vi "Tag_Value_Entry_PopUp.vi"(6 "Write Type":enum16{"SetRequest", "WriteValue"}(ring), 7 "Namespace":string, 8 "error in (no error)":errorcluster, 9 "Timeout (-1)":i32=-1, 10 "Synchronous (F)":bool, 11 "Tag Name":string) -> (0 "error out":errorcluster, 1 "found":bool, 2 "New Value":variant, 3 "Apply":bool)   [LabVIEW 2020, in "Tag Watchlist.lvlib"]
doc: "Tag value entrry pop-up. By specifying a Tag Name, the tag's value is looked up and the appropriately typed popup is launched.\n\nSelect either SetRequest or WriteValue for Write Type. Write value should be for debugging and testing purposes only. Set Request send the value by Set Request event instead of writing directly to the Tag's value.\n\nSupported Types are:\n- Boolean\n- Signed Integer\n- Unsigned Integer\n- Floating Point\n- String\n\nAny other type will launch the string value entry popup with the JSON representation of the value. BE CAREFUL."
uses:
  Tag Watchlist.lvlib
  Tag Engine.lvlib
  Tag/Tag.lvclass
  <vilib>/JDP Science/JSONtext/JSONtext.lvlib
panel:
  # "!!! Write Value is for debugging purposes only !!"
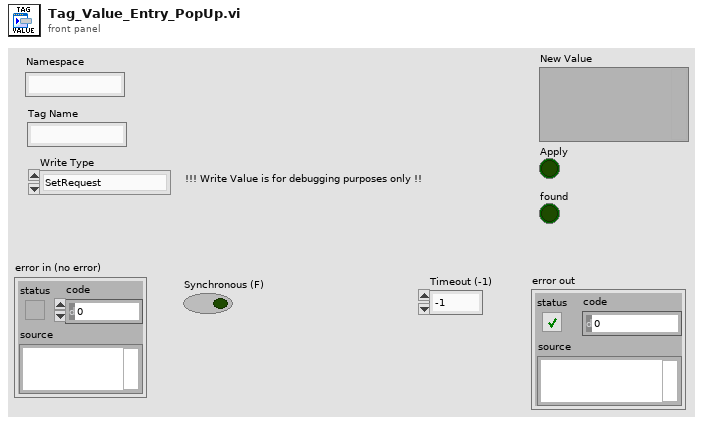
[diagram p1: front panel]
types:
  T1 = typedef "NI_Data Type.lvlib/Data Type.ctl" = enum8{"Invalid Type", "Void", "I8", "I16", "I32", "I64", "U8", "U16", "U32", "U64", "Single Float", "Double Float", "Extended Float", "Single Complex", "Double Complex", "Extended Complex", "Enum U8", "Enum U16", "Enum U32", "Enum U64", "Single Float With Unit", "Double Float With Unit", "Extended Float With Unit", "Single Complex with Unit", "Double Complex with Unit", "Extended Complex with Unit", "Boolean", "String", "Path", "Picture", "Tag", "Array", "Cluster", "Variant", "LV Variant", "Waveform", "Timestamp", "Digital Waveform", "Digital Data", "ExpressData", "Refnum", "External Data", "VI", "Poly VI", "LabVIEW Class Instance", "Fixed Point", "Set Collection", "Map Collection"}
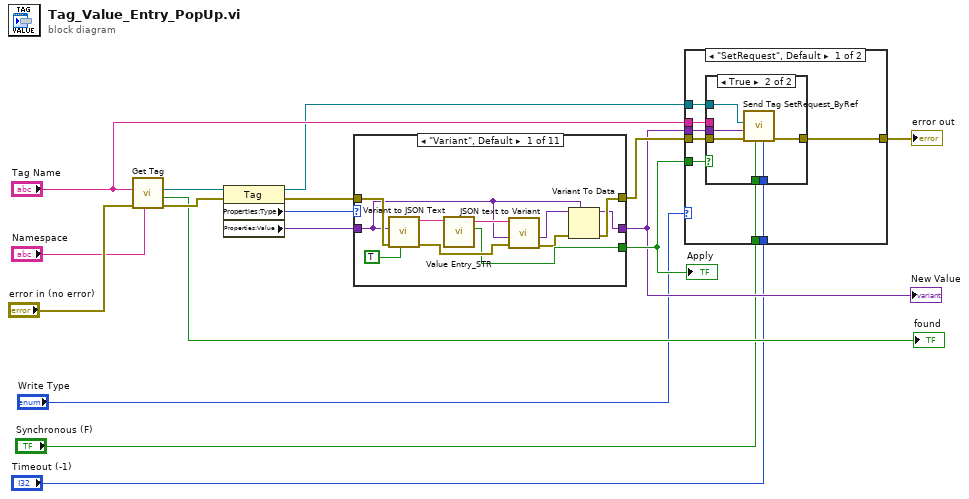
[diagram p0: block diagram]
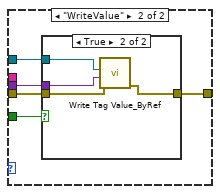
[diagram p3: hidden frame]
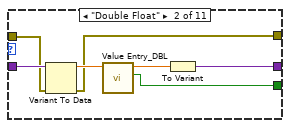
[diagram p5: hidden frame]
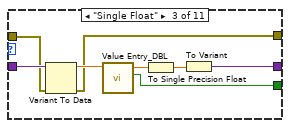
[diagram p6: hidden frame]
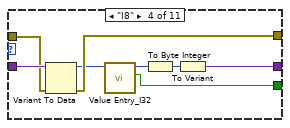
[diagram p7: hidden frame]
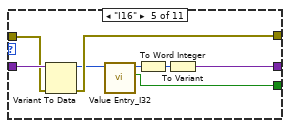
[diagram p8: hidden frame]
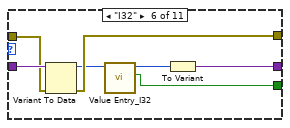
[diagram p9: hidden frame]
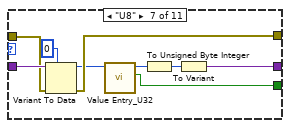
[diagram p10: hidden frame]
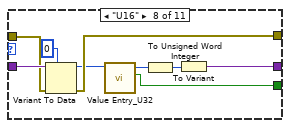
[diagram p11: hidden frame]
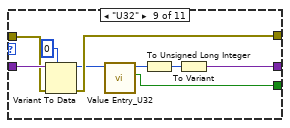
[diagram p12: hidden frame]
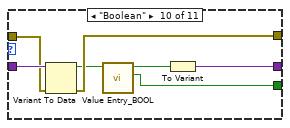
[diagram p13: hidden frame]
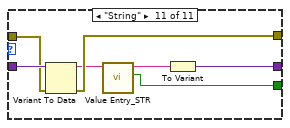
[diagram p14: hidden frame]
diagram:
  n1 = call "Get Tag.vi"("Namespace"="Namespace", "error in (no error)"="error in (no error)", "Name"="Tag Name") -> ("error out"=w7:errorcluster, "found"=→"found":bool, "Tag Ref out"=w17:refnum<data-value>)  [unwired: 6 in]
  n2 = property class="Tag"(reference=w17, error in=w7) -> (reference out=w4:refnum<data-value>, error out=w13:errorcluster, "Properties:Type"=w16:T1, "Properties:Value"=w15:variant)
  n3 = case shown="\"Variant\", Default" w16 {
    tunnel: w15 -> [w20 w35 w43 w51 w59 w66 w75 w84 w93 w100 w107]
    tunnel: w13 -> [w24 w33 w41 w50 w58 w65 w74 w83 w92 w99 w106]
    tunnel: [w21 w32 w40 w49 w57 w64 w73 w82 w91 w98 w105] -> w12
    tunnel: [w23 w30 w39 w46 w54 w61 w70 w79 w88 w94 w101] -> w11
    tunnel: [w19 w29 w38 w48 w56 w63 w72 w81 w90 w97 w104] -> w9
    frame "Variant", Default {
      n4 = call <vilib>:"Variant to JSON Text.vi"("Pretty Print?"=TRUE, "error in (no error)"=w24, "Variant"=w20) -> ("error out"=w25:errorcluster, "<JSON>"=w27:string)  [unwired: 6 in, 1 out]
      n5 = call "Value Entry_STR.vi"("Value In"=w27) -> ("Apply"=w23:bool, "Value Out"=w26:string)  [unwired: 9 in]
      n6 = call <vilib>:"JSON text to Variant.vi"("error in (no error)"=w25, "Data Type"=w20, "JSON"=w26) -> ("error out"=w22:errorcluster, "Variant out"=w18:variant)  [unwired: 7 in]
      n7 = Variant To Data(error in=w22, type=w20, Variant=w18) -> (data=w19:variant, error out=w21:errorcluster)
    }
    frame "Double Float" {
      n8 = Variant To Data(error in=w33, Variant=w35) -> (data=w34:dbl, error out=w32:errorcluster)  [unwired: 1 in]
      n9 = call "Value Entry_DBL.vi"("Value In"=w34) -> ("Apply"=w30:bool, "Value Out"=w31:dbl)  [unwired: 9 in]
      n10 = To Variant(anything=w31) -> (Variant=w29:variant)
    }
    frame "Single Float" {
      n11 = Variant To Data(error in=w41, Variant=w43) -> (data=w42:dbl, error out=w40:errorcluster)  [unwired: 1 in]
      n12 = call "Value Entry_DBL.vi"("Value In"=w42) -> ("Apply"=w39:bool, "Value Out"=w37:dbl)  [unwired: 9 in]
      n13 = To Single Precision Float(number=w37) -> (single precision float=w36:sgl)
      n14 = To Variant(anything=w36) -> (Variant=w38:variant)
    }
    frame "I8" {
      n15 = Variant To Data(error in=w50, Variant=w51) -> (data=w47:i32, error out=w49:errorcluster)  [unwired: 1 in]
      n16 = call "Value Entry_I32.vi"("Value In"=w47) -> ("Apply"=w46:bool, "Value Out"=w45:i32)  [unwired: 9 in]
      n17 = To Byte Integer(number=w45) -> (8bit integer=w44:i8)
      n18 = To Variant(anything=w44) -> (Variant=w48:variant)
    }
    frame "I16" {
      n19 = Variant To Data(error in=w58, Variant=w59) -> (data=w55:i32, error out=w57:errorcluster)  [unwired: 1 in]
      n20 = call "Value Entry_I32.vi"("Value In"=w55) -> ("Apply"=w54:bool, "Value Out"=w53:i32)  [unwired: 9 in]
      n21 = To Word Integer(number=w53) -> (16bit integer=w52:i16)
      n22 = To Variant(anything=w52) -> (Variant=w56:variant)
    }
    frame "I32" {
      n23 = Variant To Data(error in=w65, Variant=w66) -> (data=w62:i32, error out=w64:errorcluster)  [unwired: 1 in]
      n24 = call "Value Entry_I32.vi"("Value In"=w62) -> ("Apply"=w61:bool, "Value Out"=w60:i32)  [unwired: 9 in]
      n25 = To Variant(anything=w60) -> (Variant=w63:variant)
    }
    frame "U8" {
      n26 = Variant To Data(error in=w74, type=u32 0, Variant=w75) -> (data=w71:u32, error out=w73:errorcluster)
      n27 = call "Value Entry_U32.vi"("Value In"=w71) -> ("Apply"=w70:bool, "Value Out"=w67:u32)  [unwired: 9 in]
      n28 = To Unsigned Byte Integer(number=w67) -> (unsigned 8bit integer=w68:u8)
      n29 = To Variant(anything=w68) -> (Variant=w72:variant)
    }
    frame "U16" {
      n30 = Variant To Data(error in=w83, type=u32 0, Variant=w84) -> (data=w80:u32, error out=w82:errorcluster)
      n31 = call "Value Entry_U32.vi"("Value In"=w80) -> ("Apply"=w79:bool, "Value Out"=w77:u32)  [unwired: 9 in]
      n32 = To Unsigned Word Integer(number=w77) -> (unsigned 16bit integer=w76:u16)
      n33 = To Variant(anything=w76) -> (Variant=w81:variant)
    }
    frame "U32" {
      n34 = Variant To Data(error in=w92, type=u32 0, Variant=w93) -> (data=w89:u32, error out=w91:errorcluster)
      n35 = call "Value Entry_U32.vi"("Value In"=w89) -> ("Apply"=w88:bool, "Value Out"=w86:u32)  [unwired: 9 in]
      n36 = To Unsigned Long Integer(number=w86) -> (unsigned 32bit integer=w85:u32)
      n37 = To Variant(anything=w85) -> (Variant=w90:variant)
    }
    frame "Boolean" {
      n38 = Variant To Data(error in=w99, Variant=w100) -> (data=w95:bool, error out=w98:errorcluster)  [unwired: 1 in]
      n39 = call "Value Entry_BOOL.vi"("Value In"=w95) -> ("Apply"=w94:bool, "Value Out"=w96:bool)  [unwired: 9 in]
      n40 = To Variant(anything=w96) -> (Variant=w97:variant)
    }
    frame "String" {
      n41 = Variant To Data(error in=w106, Variant=w107) -> (data=w102:string, error out=w105:errorcluster)  [unwired: 1 in]
      n42 = call "Value Entry_STR.vi"("Value In"=w102) -> ("Apply"=w101:bool, "Value Out"=w103:string)  [unwired: 9 in]
      n43 = To Variant(anything=w103) -> (Variant=w104:variant)
    }
  }
  "New Value" <- w9
  "Apply" <- w11
  n44 = case shown="\"SetRequest\", Default" "Write Type" {
    tunnel: "Tag Name" -> [w115 _]
    tunnel: w12 -> [w114 w126]
    tunnel: w11 -> [w113 w127]
    tunnel: [w112 w123] -> w10
    tunnel: w9 -> [w111 w125]
    tunnel: w4 -> [w108 w124]
    tunnel: "Synchronous (F)" -> [w110 _]
    tunnel: "Timeout (-1)" -> [w109 _]
    frame "SetRequest", Default {
      n45 = case shown="True" w113 {
        tunnel: w115 -> [_ _]
        tunnel: w114 -> [w116 w122]
        tunnel: [w116 w121] -> w112
        tunnel: w111 -> [_ w120]
        tunnel: w110 -> [_ w119]
        tunnel: w109 -> [_ w118]
        tunnel: w108 -> [_ w117]
        frame False {
        }
        frame True {
          n46 = call "Send Tag SetRequest_ByRef.vi"("Timeout (-1)"=w118, "Synchronous (F)"=w119, "error in (no error)"=w122, "Value"=w120, "Tag Ref in"=w117) -> ("error out"=w121:errorcluster)  [unwired: 4 in, 2 out]
        }
      }
    }
    frame "WriteValue" {
      n47 = case shown="True" w127 {
        tunnel: w126 -> [w128 w130]
        tunnel: w125 -> [_ w131]
        tunnel: w124 -> [_ w132]
        tunnel: [w128 w129] -> w123
        frame False {
        }
        frame True {
          n48 = call "Write Tag Value_ByRef.vi"("error in (no error)"=w130, "Value"=w131, "Tag Ref in"=w132) -> ("error out"=w129:errorcluster)  [unwired: 7 in, 1 out]
        }
      }
    }
  }
  "error out" <- w10
